vi "libssh2_knownhost_writeline.vi"(7 "buffer length (4096)":u32=4096, 8 "error in (no error)":errorcluster, 9 "type (OpenSSH)":T2, 10 "host key":T1, 11 "host key database":T3) -> (0 "error out":errorcluster, 2 "line":string)   [LabVIEW 2017, in "libssh2.lvlib"]
doc: "Write a host key to a string."
uses:
  libssh2.lvlib
  Host Key Database Refnum.ctl
  Host Key File Type.ctl
  Host Key Refnum.ctl
  Not A Host Key Database.vi
  <vilib>/Utility/error.llb/Error Cluster From Error Code.vi
  Not A Host Key.vi
  Global Settings.vi
  Read Host Key Database Refnum.vi
  <vilib>/Utility/semaphor.llb/Acquire Semaphore.vi
  <vilib>/Utility/semaphor.llb/Release Semaphore.vi
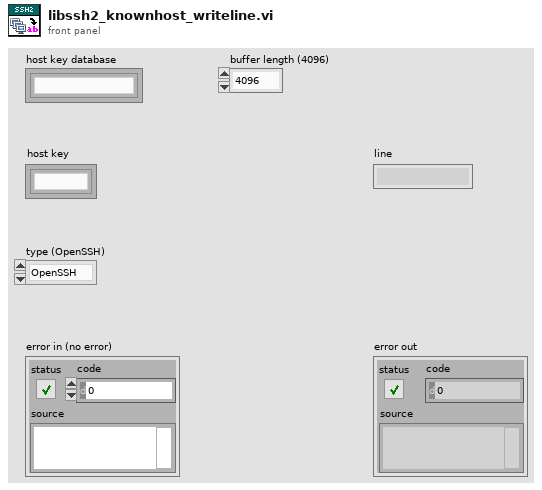
[diagram p1: front panel]
types:
  T1 = typedef "libssh2.lvlib/Host Key Refnum.ctl" = refnum<k1>
  T2 = typedef "libssh2.lvlib/Host Key File Type.ctl" = enum16{"OpenSSH"}
  T3 = typedef "libssh2.lvlib/Host Key Database Refnum.ctl" = refnum<k1>
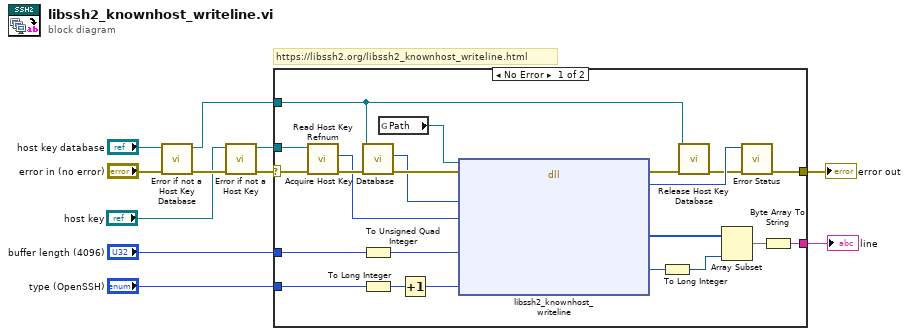
[diagram p0: block diagram]
diagram:
  # "https://libssh2.org/libssh2_knownhost_writeline.html"
  n1 = call "Error if not a Host Key Database.vi"("error in (no error)"="error in (no error)", "host key database"="host key database") -> ("error out"=w8:errorcluster, "host key database out"=w6:T3)  [unwired: 8 in]
  n2 = call "Error if not a Host Key.vi"("error in (no error)"=w8, "host key"="host key") -> ("error out"=w3:errorcluster, "host key out"=w1:T1)  [unwired: 8 in]
  n3 = case shown="No Error" w3 {
    selector: w3 -> [w32 w34]
    tunnel: [w31 w34] -> w11
    tunnel: "type (OpenSSH)" -> [w33 _]
    tunnel: w6 -> [w12 _]
    tunnel: "buffer length (4096)" -> [w23 _]
    tunnel: [w19 _] -> w4
    tunnel: w1 -> [w16 _]
    frame No Error {
      n4 = call "Read Host Key Refnum.vi"("error in (no error)"=w32, "host key"=w16) -> ("error out"=w18:errorcluster, "libssh2_knownhost*"=w17:u64)  [unwired: 7 in, 1 out]
      n5 = call "Acquire Host Key Database.vi"("error in (no error)"=w18, "host key database"=w12) -> ("error out"=w29:errorcluster, "LIBSSH2_KNOWNHOSTS*"=w28:u64)  [unwired: 8 in]
      n6 = To Unsigned Quad Integer(1:w23) -> (0:w14:u64)
      n7 = To Long Integer(number=w33) -> (32bit integer=w25:i32)
      n8 = global read "Global Settings.vi" "Path"() -> (w27:path)
      n9 = Increment(x=w25) -> (x+1=w24:i32)
      n10 = dll-call lib="?" fn="libssh2_knownhost_writeline"(path in=w27, error in=w29, "hosts"=w28, "known"=w17, "buflen"=w14, "type"=w24) -> (error out=w30:errorcluster, "return value"=w26:i32, "buffer"=w22:u8[], "outlen"=w21:u64)  [unwired: 7 in, 1 out]
      n11 = To Long Integer(number=w21) -> (32bit integer=w15:i32)
      n12 = call "Release Host Key Database.vi"("error in (no error)"=w30, "host key database"=w12) -> ("error out"=w13:errorcluster)  [unwired: 9 in]
      n13 = Array Subset(array=w22, length=w15) -> (w20:u8[])  [unwired: 1 in]
      n14 = call "Error Status.vi"("error in (no error)"=w13, "return value"=w26) -> ("error out"=w31:errorcluster)  [unwired: 8 in, 1 out]
      n15 = Byte Array To String(unsigned byte array=w20) -> (string=w19:string)
    }
    frame Error {
    }
  }
  "error out" <- w11
  "line" <- w4
